vi "Add Argument.vi"(7 "Prepend? (F = Append)":bool, 9 "error in (no error)":errorcluster, 10 "argument data":string, 11 "argument":string) -> (1 "error out":errorcluster)   [LabVIEW 2019, in "Error Generation.lvlib"]
doc: "Add or replace the argument and data to the error cluster, if error or warning.\n- - -\nCopyright (c) 2023, Merecs Engineering GmbH"
uses:
  Error Generation.lvlib
panel:
  # "Connector Pane"
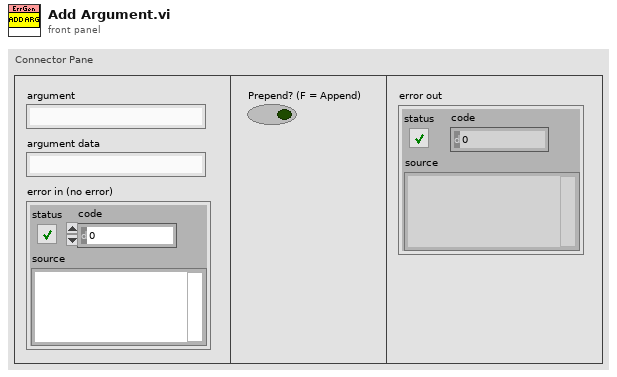
[diagram p1: front panel]
types:
  T1 = typedef "TagReturnType.ctl" = enum16{"No Tag", "<err>", "<append>"}
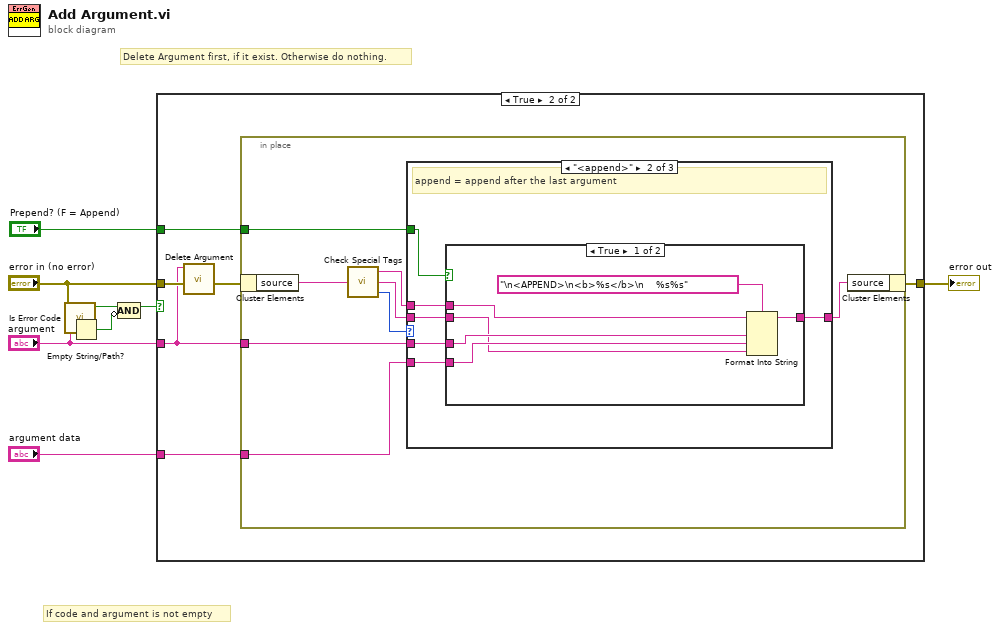
[diagram p0: block diagram]
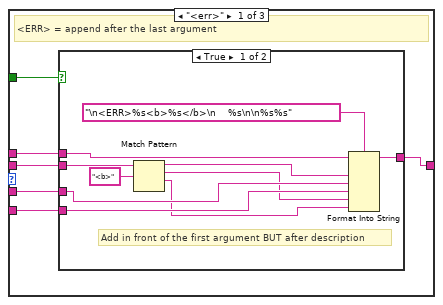
[diagram p3: hidden frame]
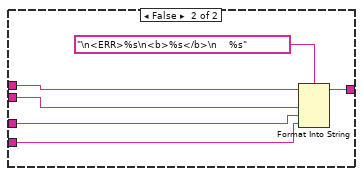
[diagram p4: hidden frame]
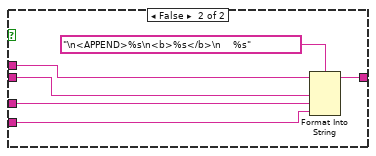
[diagram p5: hidden frame]
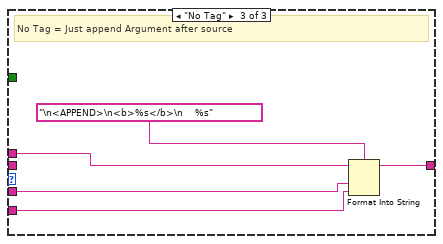
[diagram p6: hidden frame]
diagram:
  # "If code and argument is not empty"
  # "Delete Argument first, if it exist. Otherwise do nothing."
  n1 = call "Is Error Code.vi"("error in (no error)"="error in (no error)") -> ("Code!=0"=w8:bool)  [unwired: 5 in, 1 out]
  n2 = Empty String/Path?(string/path="argument") -> (empty?=w2:bool)
  n3 = Compound Arithmetic op=AND(w8, invert w2) -> (w3:bool)
  n4 = case shown="True" w3 {
    tunnel: [w9 w14] -> w5
    tunnel: "error in (no error)" -> [w9 w15]
    tunnel: "argument" -> [_ w11]
    tunnel: "argument data" -> [_ w12]
    tunnel: "Prepend? (F = Append)" -> [_ w10]
    frame False {
    }
    frame True {
      n5 = call "Delete Argument.vi"("error in (no error)"=w15, "argument"=w11) -> ("error out"=w13:errorcluster)  [unwired: 8 in, 1 out]
      n6 = in-place {
        in-place-border: w11 -> [w18]
        in-place-border: w12 -> [w17]
        in-place-border: w10 -> [w16]
        n7 = in-place-cluster #1(w13) -> ("source"=w20:string)
        n8 = call <vilib>:"Check Special Tags.vi"("source"=w20) -> ("Before Tag (source)"=w21:string, "After Tag (special data)"=w22:string, "Tag Found?"=w23:T1)
        n9 = case shown="\"<append>\"" w23 {
          tunnel: w22 -> [w25 w47 _]
          tunnel: w18 -> [w29 w51 w67]
          tunnel: [w28 w50 w66] -> w19
          tunnel: w17 -> [w27 w49 w65]
          tunnel: w21 -> [w26 w48 w64]
          tunnel: w16 -> [w24 w46 _]
          frame "<err>" {
            # "<ERR> = append after the last argument"
            n10 = case shown="True" w24 {
              tunnel: w29 -> [w33 w44]
              tunnel: [w38 w43] -> w28
              tunnel: w27 -> [w32 w42]
              tunnel: w26 -> [w37 w41]
              tunnel: w25 -> [w35 w40]
              frame True {
                # "Add in front of the first argument BUT after description"
                n11 = Match Pattern(string=w35, regular expression="<b>") -> (before substring=w34:string, match substring=w31:string, after substring=w30:string)  [unwired: 1 in, 1 out]
                n12 = Format Into String(format string="\n<ERR>%s<b>%s</b>\n    %s\n\n%s%s", initial string=w37, w34, w33, w32, w31, w30) -> (resulting string=w38:string)  [unwired: 1 in, 1 out]
              }
              frame False {
                n13 = Format Into String(format string="\n<ERR>%s\n<b>%s</b>\n    %s", initial string=w41, w40, w44, w42) -> (resulting string=w43:string)  [unwired: 1 in, 1 out]
              }
            }
          }
          frame "<append>" {
            # "append = append after the last argument"
            n14 = case shown="True" w46 {
              tunnel: w51 -> [w56 w62]
              tunnel: [w55 w61] -> w50
              tunnel: w49 -> [w54 w60]
              tunnel: w48 -> [w53 w59]
              tunnel: w47 -> [w52 w58]
              frame True {
                n15 = Format Into String(format string="\n<APPEND>\n<b>%s</b>\n    %s%s", initial string=w53, w56, w54, w52) -> (resulting string=w55:string)  [unwired: 1 in, 1 out]
              }
              frame False {
                n16 = Format Into String(format string="\n<APPEND>%s\n<b>%s</b>\n    %s", initial string=w59, w58, w62, w60) -> (resulting string=w61:string)  [unwired: 1 in, 1 out]
              }
            }
          }
          frame "No Tag" {
            # "No Tag = Just append Argument after source"
            n17 = Format Into String(format string="\n<APPEND>\n<b>%s</b>\n    %s", initial string=w64, w67, w65) -> (resulting string=w66:string)  [unwired: 1 in, 1 out]
          }
        }
        n18 = in-place-cluster #1("source"=w19) -> (w14:errorcluster)
      }
    }
  }
  "error out" <- w5
